vi "Lab_2_Calculate_HR_Zones.vi"(8 "error in (no error)":errorcluster, 11 "HR Data Structure IN":T1) -> (0 "error out":errorcluster, 3 "HR Data Structure OUT":T1)   [LabVIEW 2025]
uses:
  <vilib>/Analysis/NI_AALBase.lvlib
  <vilib>/Analysis/baseanly.llb/Mean (DBL).vi
  raw_data.ctl
  runners_data.ctl
  hr_data_structure.ctl
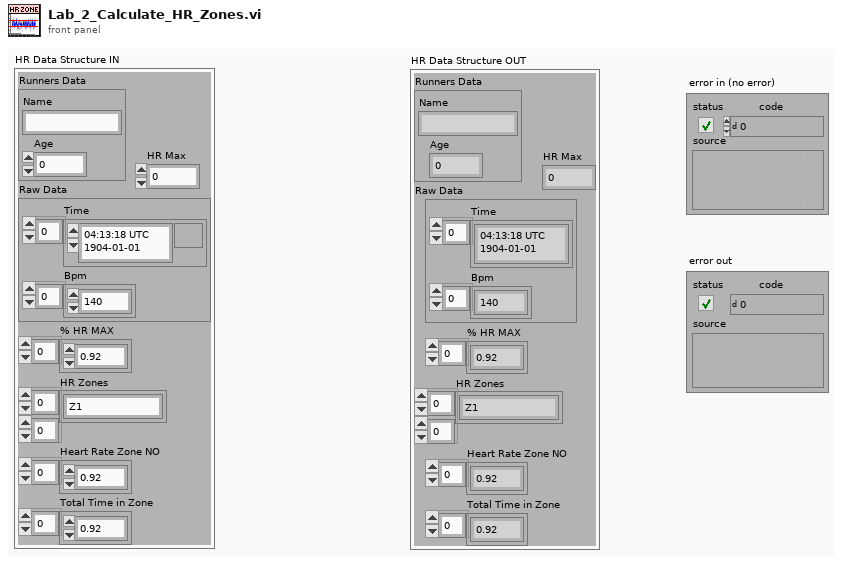
[diagram p1: front panel]
types:
  T1 = typedef "hr_data_structure.ctl" = cluster{"Runners Data":T2, "Raw Data":T3, "% HR MAX ":dbl[], "HR Zones":string[][], "Heart Rate Zone NO":dbl[], "Total Time in Zone":dbl[], "HR Max":dbl}
  T2 = typedef "runners_data.ctl" = cluster{"Name":string, "Age":i32}
  T3 = typedef "raw_data.ctl" = cluster{"Time":timestamp[], "Bpm":i32[]}
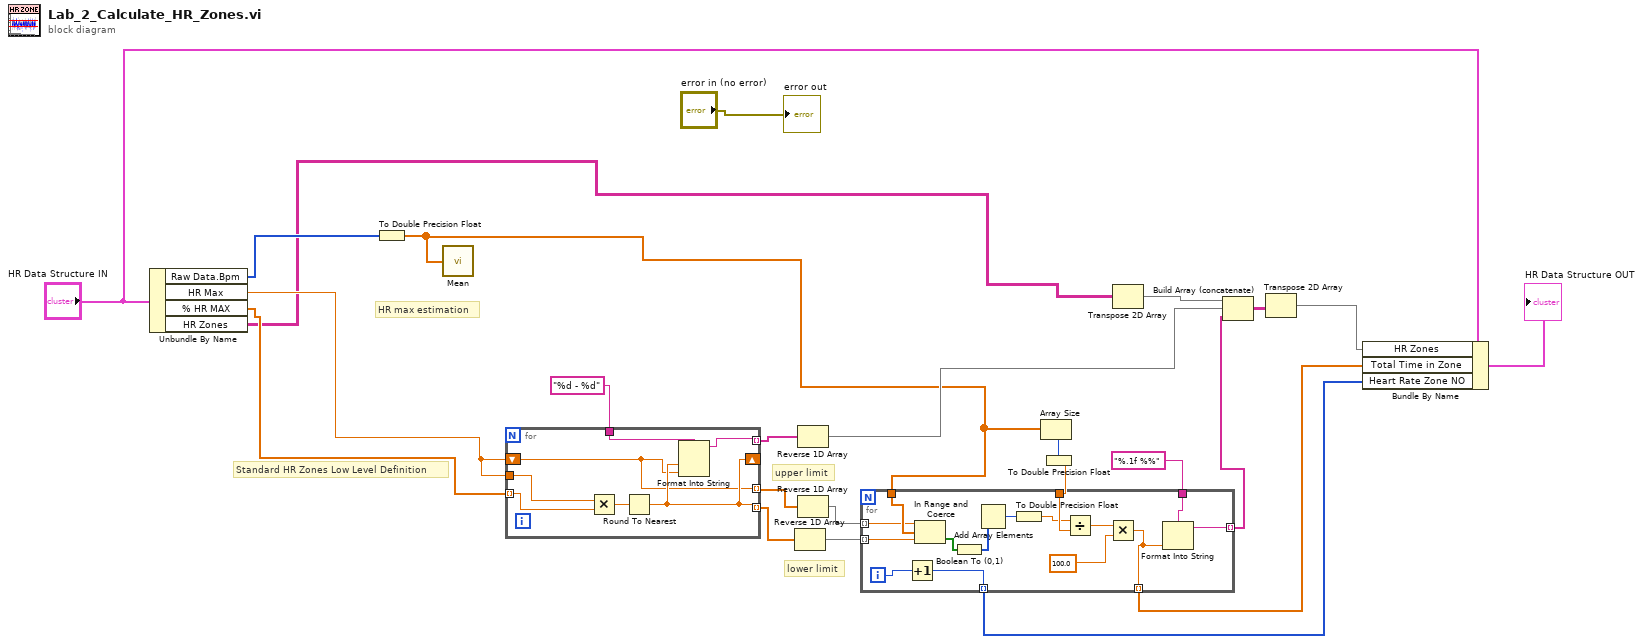
[diagram p0: block diagram]
diagram:
  # "upper limit"
  # "lower limit"
  # "Standard HR Zones Low Level Definition"
  # "HR max estimation"
  n1 = Unbundle By Name("HR Data Structure IN") -> ("Raw Data.Bpm"=w8:i32[], "HR Max"=w9:dbl, "% HR MAX"=w10:dbl[], "HR Zones"=w7:string[][])
  n2 = To Double Precision Float(number=w8) -> (double precision float=w12:dbl[])
  n3 = call-poly <vilib>:"Mean.vi"("X"=w12) -> ()  [unwired: 2 out]
  n4 = for {
    tunnel: w10 -> [w31] mode=indexing
    shift-right: [w26] -> _
    shift-left: w9 -> [w25]
    tunnel: w9 -> [w29]
    tunnel: "%d - %d" -> [w28]
    tunnel: [w27] -> w23 mode=indexing
    tunnel: [w26] -> w15 mode=indexing
    tunnel: [w25] -> w16 mode=indexing
    n5 = Multiply(x=w29, y=w31) -> (x*y=w30:dbl)
    n6 = Round To Nearest(number=w30) -> (nearest integer value=w26:dbl)
    n7 = Format Into String(format string=w28, w26, w25) -> (resulting string=w27:string)  [unwired: 2 in, 1 out]
  }
  n8 = Reverse 1D Array(array=w15) -> (reversed array=w13:dbl[])
  n9 = Reverse 1D Array(array=w23) -> (reversed array=w20:string[])
  n10 = Reverse 1D Array(array=w16) -> (reversed array=w14:dbl[])
  n11 = Array Size(array=w12) -> (size(s)=w22:i32)
  n12 = To Double Precision Float(number=w22) -> (double precision float=w11:dbl)
  n13 = for {
    tunnel: w12 -> [w45]
    tunnel: w11 -> [w42]
    tunnel: "%.1f %%" -> [w39]
    tunnel: [w38] -> w18 mode=indexing
    tunnel: [w37] -> w3 mode=indexing
    tunnel: [w34] -> w2 mode=indexing
    tunnel: w14 -> [w36] mode=indexing
    tunnel: w13 -> [w35] mode=indexing
    i -> [w34]
    n14 = Increment(x=w34) -> ()  [unwired: 1 out]
    n15 = In Range and Coerce(upper limit=w36, x=w45, lower limit=w35) -> (In Range?=w44:bool[])  [unwired: 1 out]
    n16 = Boolean To (0,1)(Boolean=w44) -> (0, 1=w43:i16[])
    n17 = Add Array Elements(numeric array=w43) -> (sum=w41:i16)
    n18 = To Double Precision Float(number=w41) -> (double precision float=w33:dbl)
    n19 = Divide(x=w33, y=w42) -> (x/y=w40:dbl)
    n20 = Multiply(x=w40, y=100.0) -> (x*y=w37:dbl)
    n21 = Format Into String(format string=w39, w37) -> (resulting string=w38:string)  [unwired: 2 in, 1 out]
  }
  n22 = Transpose 2D Array(2D array=w7) -> (transposed array=w19:string[][])
  n23 = Build Array (concatenate)(w19, w20, w18) -> (w17:string[][])
  n24 = Transpose 2D Array(2D array=w17) -> (transposed array=w4:string[][])
  n25 = Bundle By Name(cluster="HR Data Structure IN", "HR Zones"=w4, "Total Time in Zone"=w3, "Heart Rate Zone NO"=w2) -> (→"HR Data Structure OUT":T1)
  "error out" <- "error in (no error)"
